vi "Game_Click.vi"(0 "Context":T1={"Screen"=enum."Settings", "Settings"=[0, 0, 1, 1], "Board"={"Grid"=array15x15[225 elements], "Move History"=[], "Last Move"={"Row"=-1, "Col"=-1, "Stone"=enum."Empty"}}, "Status"=enum."Idle", "Game ID"=0, "Player Stone"=enum."Black", "Hover"={"Row"=-1, "Col"=-1, "Stone"=enum."Empty"}, "Hover Button"=-1, "Win Line"=[], "Score 1"=0, "Score 2"=0, "Draws"=0, "Status Text"="", "Status Color"=0}, 5 "X":i32, 7 "Y":i32, 11 "error in":errorcluster) -> (4 "Context out":T1={"Screen"=enum."Settings", "Settings"=[0, 0, 1, 1], "Board"={"Grid"=array15x15[225 elements], "Move History"=[], "Last Move"={"Row"=-1, "Col"=-1, "Stone"=enum."Empty"}}, "Status"=enum."Idle", "Game ID"=0, "Player Stone"=enum."Black", "Hover"={"Row"=-1, "Col"=-1, "Stone"=enum."Empty"}, "Hover Button"=-1, "Win Line"=[], "Score 1"=0, "Score 2"=0, "Draws"=0, "Status Text"="", "Status Color"=0}, 6 "Need AI":bool, 15 "error out":errorcluster)   [LabVIEW 2026]
doc: "마우스 클릭 (X,Y) 처리. 설정 화면: 모드/선공/난이도/규칙 선택, 게임 시작.\n게임 화면: 무르기/새 게임/설정 버튼, 그 외는 바둑판 착수. Need AI = AI에게 계산 요청 필요."
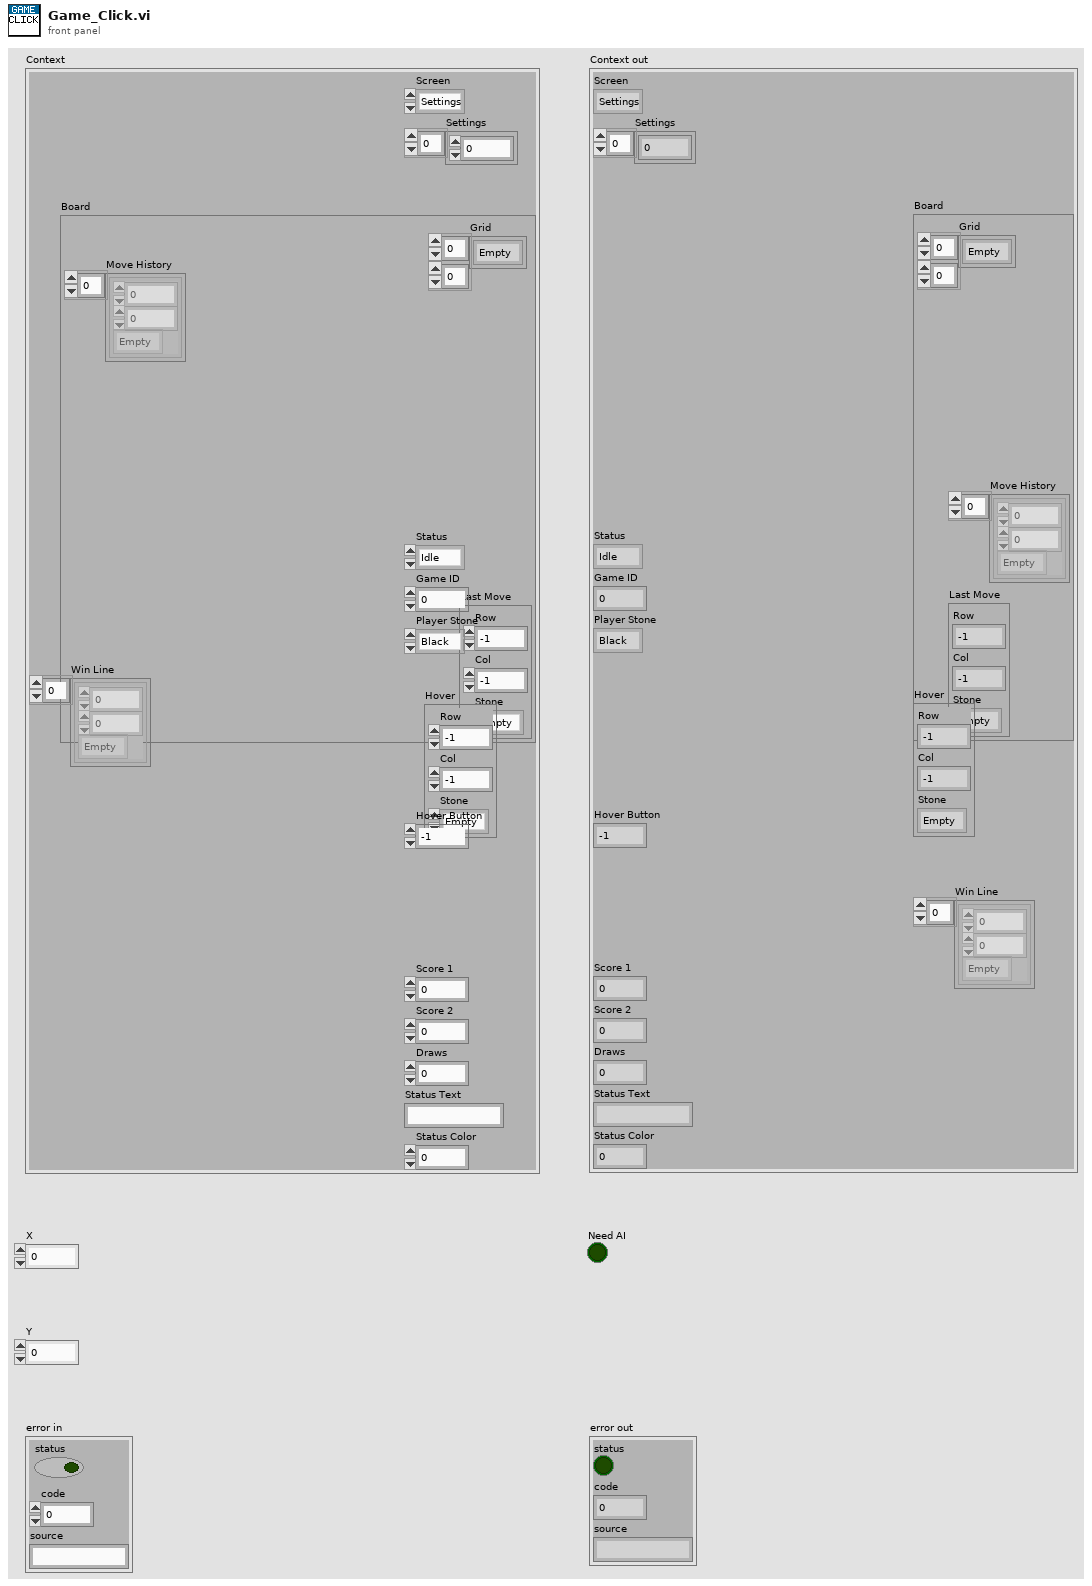
[diagram p1: front panel]
types:
  T1 = cluster{"Screen":enum16{"Settings", "Game"}, "Settings":i32[], "Board":cluster{"Grid":enum8{"Empty", "Black", "White"}[][], "Move History":cluster{"Row":i32, "Col":i32, "Stone":enum8{"Empty", "Black", "White"}}[], "Last Move":cluster{"Row":i32, "Col":i32, "Stone":enum8{"Empty", "Black", "White"}}}, "Status":enum16{"Idle", "Player Turn", "AI Thinking", "Game Over"}, "Game ID":u32, "Player Stone":enum8{"Empty", "Black", "White"}, "Hover":cluster{"Row":i32, "Col":i32, "Stone":enum8{"Empty", "Black", "White"}}, "Hover Button":i32, "Win Line":cluster{"Row":i32, "Col":i32, "Stone":enum8{"Empty", "Black", "White"}}[], "Score 1":i32, "Score 2":i32, "Draws":i32, "Status Text":string, "Status Color":u32}
  T2 = enum16{"Idle", "Player Turn", "AI Thinking", "Game Over"}
  T3 = cluster{"Rect":cluster{"left":i16, "top":i16, "right":i16, "bottom":i16}, "Fill":u32, "Fill Sel":u32, "Border":u32, "Border Sel":u32, "Text":string, "Text Color":u32, "Text Sel":u32, "Size":i16, "Bold":bool, "Group":i32, "Value":i32, "Radius":i16}[]
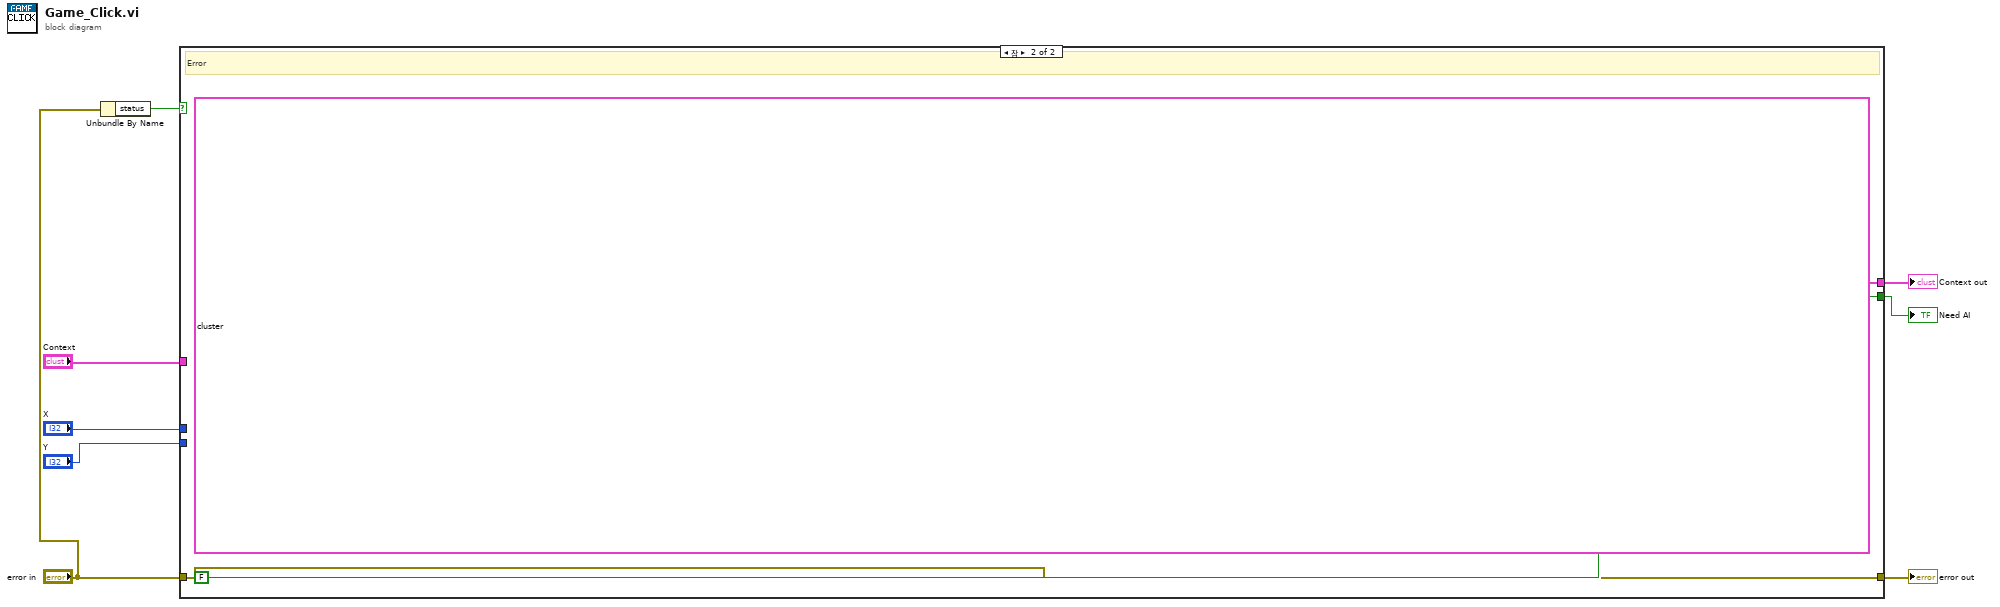
[diagram p0: block diagram]
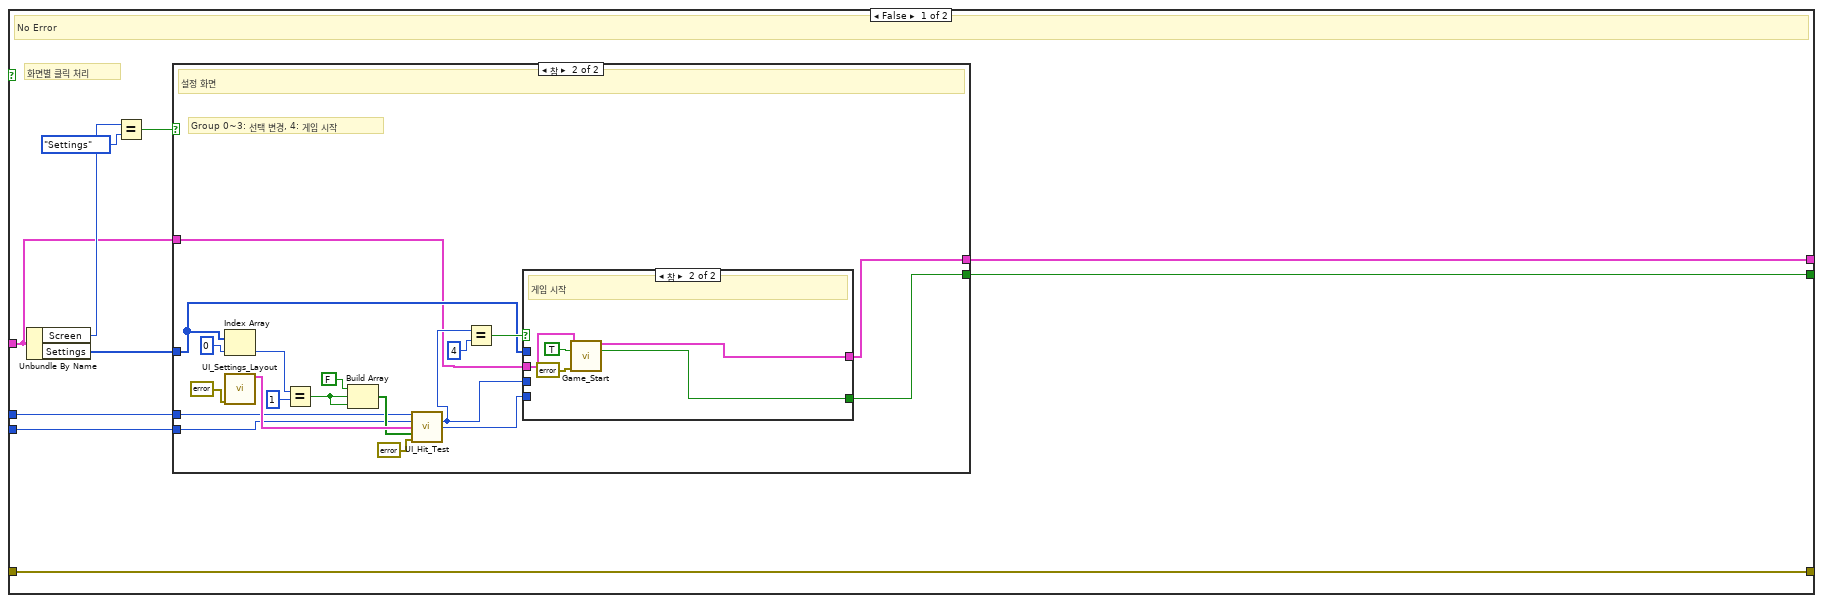
[diagram p2: hidden frame]
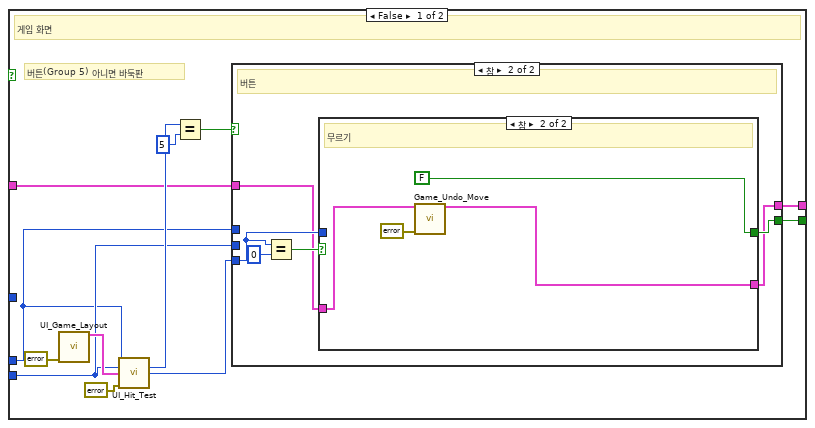
[diagram p3: hidden frame]
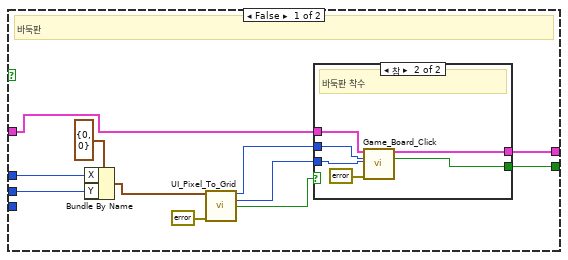
[diagram p4: hidden frame]
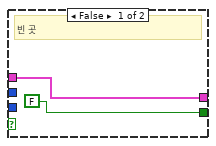
[diagram p5: hidden frame]
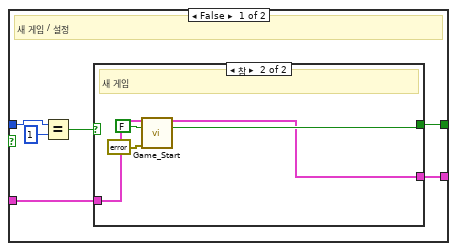
[diagram p6: hidden frame]
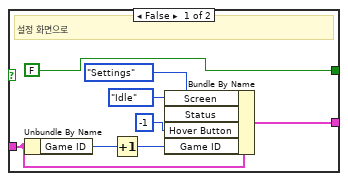
[diagram p7: hidden frame]
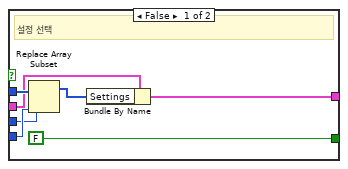
[diagram p8: hidden frame]
diagram:
  n1 = Unbundle By Name("error in") -> ("status"=w5:bool)
  n2 = case shown="참" w5 {
    tunnel: "Context" -> [w9 _]
    tunnel: "X" -> [w10 _]
    tunnel: "Y" -> [w11 _]
    tunnel: "error in" -> [w12 w110]
    tunnel: [w12 w110] -> w8
    tunnel: [w17 T1 {"Screen"=enum."Settings", "Settings"=[0, 0, 1, 1], "Board"={"Grid"=array15x15[225 elements], "Move History"=[], "Last Move"={"Row"=-1, "Col"=-1, "Stone"=enum."Empty"}}, "Status"=enum."Idle", "Game ID"=0, "Player Stone"=enum."Black", "Hover"={"Row"=-1, "Col"=-1, "Stone"=enum."Empty"}, "Hover Button"=-1, "Win Line"=[], "Score 1"=0, "Score 2"=0, "Draws"=0, "Status Text"="", "Status Color"=0}] -> w6
    tunnel: [w18 FALSE] -> w7
    frame False {
      # "화면별 클릭 처리"
      # "No Error"
      n3 = Unbundle By Name(w9) -> ("Screen"=w13:enum16{"Settings", "Game"}, "Settings"=w14:i32[])
      n4 = Equal?(x=w13, y=enum16{"Settings", "Game"}."Settings") -> (x = y?=w16:bool)
      n5 = case shown="참" w16 {
        tunnel: w9 -> [w19 w79]
        tunnel: w10 -> [w20 w80]
        tunnel: w11 -> [w21 w81]
        tunnel: w14 -> [_ w82]
        tunnel: [w29 w96] -> w17
        tunnel: [w30 w97] -> w18
        frame False {
          # "버튼(Group 5) 아니면 바둑판"
          # "게임 화면"
          n6 = call "UI_Game_Layout.vi"("error in"=errorcluster {"status"=FALSE, "code"=0, "source"=""}) -> ("Specs"=w23:T3)  [unwired: 13 in, 1 out]
          n7 = call "UI_Hit_Test.vi"("X"=w20, "Y"=w21, "Specs"=w23, "error in"=errorcluster {"status"=FALSE, "code"=0, "source"=""}) -> ("Group"=w25:i32, "Value"=w26:i32)  [unwired: 8 in, 2 out]
          n8 = Equal?(x=w25, y=5) -> (x = y?=w28:bool)
          n9 = case shown="참" w28 {
            tunnel: [w41 w55] -> w30
            tunnel: w19 -> [w31 w50]
            tunnel: w20 -> [w32 _]
            tunnel: w21 -> [w33 _]
            tunnel: w26 -> [_ w51]
            tunnel: [w40 w54] -> w29
            frame False {
              # "바둑판"
              n10 = Bundle By Name(cluster=cluster{"X":i32, "Y":i32} {"X"=0, "Y"=0}, "X"=w32, "Y"=w33) -> (w35:cluster{"X":i32, "Y":i32})
              n11 = call "UI_Pixel_To_Grid.vi"("Coords"=w35, "error in"=errorcluster {"status"=FALSE, "code"=0, "source"=""}) -> ("Row"=w37:i32, "Col"=w38:i32, "Valid"=w39:bool)  [unwired: 10 in, 1 out]
              n12 = case shown="참" w39 {
                tunnel: w31 -> [w42 w44]
                tunnel: w37 -> [_ w45]
                tunnel: w38 -> [_ w46]
                tunnel: [w42 w48] -> w40
                tunnel: [FALSE w49] -> w41
                frame False {
                  # "빈 곳"
                }
                frame True {
                  # "바둑판 착수"
                  n13 = call "Game_Board_Click.vi"("Context"=w44, "Row"=w45, "Col"=w46, "error in"=errorcluster {"status"=FALSE, "code"=0, "source"=""}) -> ("Context out"=w48:T1, "Need AI"=w49:bool)  [unwired: 9 in, 1 out]
                }
              }
            }
            frame True {
              # "버튼"
              n14 = Equal?(x=w51, y=0) -> (x = y?=w53:bool)
              n15 = case shown="참" w53 {
                tunnel: [w61 FALSE] -> w55
                tunnel: w50 -> [w56 w75]
                tunnel: w51 -> [w57 _]
                tunnel: [w60 w77] -> w54
                frame False {
                  # "새 게임 / 설정"
                  n16 = Equal?(x=w57, y=1) -> (x = y?=w59:bool)
                  n17 = case shown="참" w59 {
                    tunnel: w56 -> [w62 w70]
                    tunnel: [w68 w73] -> w60
                    tunnel: [FALSE w74] -> w61
                    frame False {
                      # "설정 화면으로"
                      n18 = Unbundle By Name(w62) -> ("Game ID"=w63:u32)
                      n19 = Increment(x=w63) -> (x+1=w67:u32)
                      n20 = Bundle By Name(cluster=w62, "Screen"=enum16{"Settings", "Game"}."Settings", "Status"=T2."Idle", "Hover Button"=-1, "Game ID"=w67) -> (w68:T1)
                    }
                    frame True {
                      # "새 게임"
                      n21 = call "Game_Start.vi"("Context"=w70, "Reset Scores"=FALSE, "error in"=errorcluster {"status"=FALSE, "code"=0, "source"=""}) -> ("Context out"=w73:T1, "Need AI"=w74:bool)  [unwired: 10 in, 1 out]
                    }
                  }
                }
                frame True {
                  # "무르기"
                  n22 = call "Game_Undo_Move.vi"("Context"=w75, "error in"=errorcluster {"status"=FALSE, "code"=0, "source"=""}) -> ("Context out"=w77:T1)  [unwired: 12 in, 1 out]
                }
              }
            }
          }
        }
        frame True {
          # "Group 0~3: 선택 변경, 4: 게임 시작"
          # "설정 화면"
          n23 = Index Array(array=w82, index=0) -> (element=w84:i32)
          n24 = call "UI_Settings_Layout.vi"("error in"=errorcluster {"status"=FALSE, "code"=0, "source"=""}) -> ("Specs"=w90:T3)  [unwired: 13 in, 1 out]
          n25 = Equal?(x=w84, y=1) -> (x = y?=w86:bool)
          n26 = Build Array(FALSE, w86, w86) -> (w88:bool[])
          n27 = call "UI_Hit_Test.vi"("X"=w80, "Y"=w81, "Specs"=w90, "Dim Groups"=w88, "error in"=errorcluster {"status"=FALSE, "code"=0, "source"=""}) -> ("Group"=w92:i32, "Value"=w93:i32)  [unwired: 7 in, 2 out]
          n28 = Equal?(x=w92, y=4) -> (x = y?=w95:bool)
          n29 = case shown="참" w95 {
            tunnel: w79 -> [w98 w105]
            tunnel: w82 -> [w99 _]
            tunnel: [w103 w108] -> w96
            tunnel: [FALSE w109] -> w97
            tunnel: w92 -> [w100 _]
            tunnel: w93 -> [w101 _]
            frame False {
              # "설정 선택"
              n30 = Replace Array Subset(array=w99, new element=w101, index=w100) -> (w102:i32[])
              n31 = Bundle By Name(cluster=w98, "Settings"=w102) -> (w103:T1)
            }
            frame True {
              # "게임 시작"
              n32 = call "Game_Start.vi"("Context"=w105, "Reset Scores"=TRUE, "error in"=errorcluster {"status"=FALSE, "code"=0, "source"=""}) -> ("Context out"=w108:T1, "Need AI"=w109:bool)  [unwired: 10 in, 1 out]
            }
          }
        }
      }
    }
    frame True {
      # "Error"
    }
  }
  "Context out" <- w6
  "Need AI" <- w7
  "error out" <- w8
